vi "simple_continous_read.vi"() -> ()   [LabVIEW 2013]
doc: "This example illustrate how to use some of the VI included in the OpenBCI toolbox"
uses:
  Comm Protocol/Control Def/channel_count.ctl
panel:
  out "CH1":dbl[](graph)
  in  "channel_count(8)":T1
  out "sample count":dbl[](graph)
  in  "stop":bool
  out "EEG Waveform Channels 1 - 8":dbl[][](graph)
  out "Console":string
  in  "COM port":refnum<visa-resource-name>
  # "Instructions:\nBefore running the VI\n1. Select the COM port for the OpenBCI receiver\n2. Select the number of channels in your board\n3. Run the VI\n4. The Device initial response is shown in the Console textbox  \n5. Click on \"Stop\" to stop the EEG acquisition"
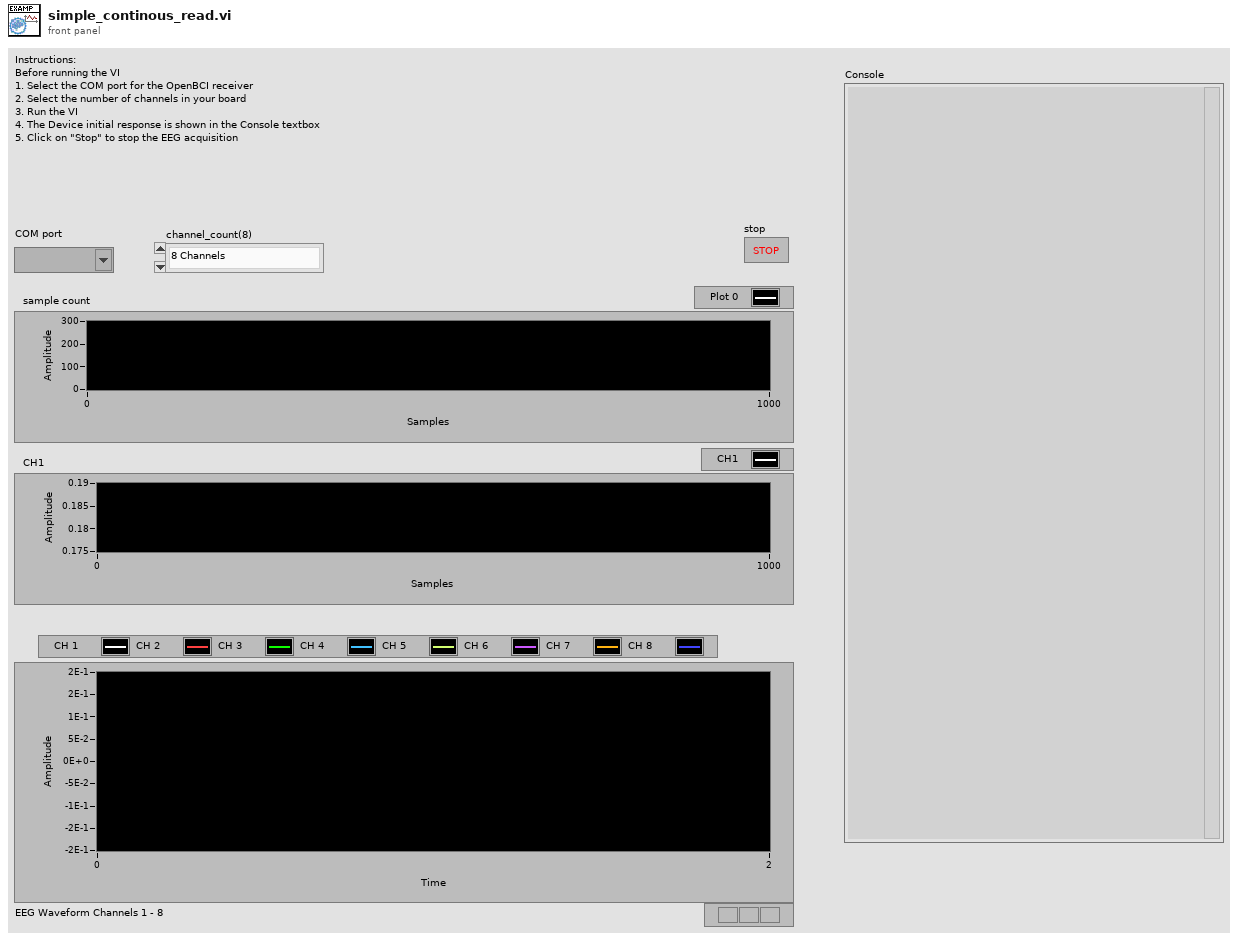
[diagram p1: front panel]
types:
  T1 = typedef "channel_count.ctl" = enum16{"8 Channels", "16 Channels"}
  T2 = typedef "openbci_device.ctl" = cluster{"COM port":refnum<visa-resource-name>, "n_ch (8)":T1, "delay_tx":u32}
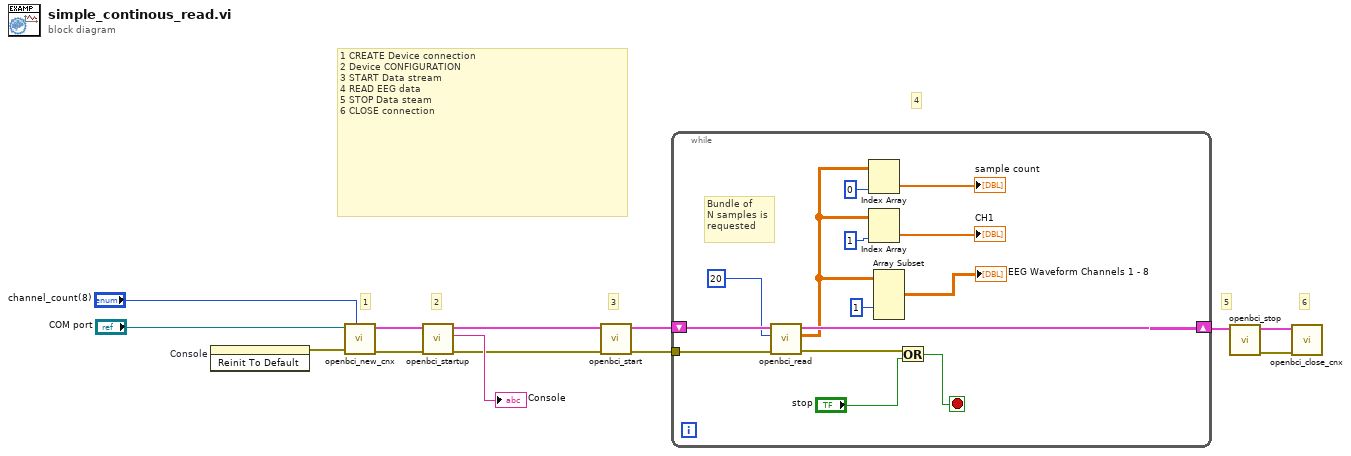
[diagram p0: block diagram]
diagram:
  # "1"
  # "4"
  # "6"
  # "5"
  # "3"
  # "2"
  # "1 CREATE Device connection\n2 Device CONFIGURATION\n3 START Data stream \n4 READ EEG data\n5 STOP Data steam\n6 CLOSE connection"
  n1 = invoke on="Console" class="Str" method="Reinit To Default"() -> (error out=w1:errorcluster)  [unwired: 3 in, 2 out]
  n2 = call "openbci_new_cnx.vi"("channel_count(8)"="channel_count(8)", "error in (no error)"=w1, "COM port"="COM port") -> ("error out"=w8:errorcluster, "OBCI dev out"=w5:T2)  [unwired: 7 in]
  n3 = call "openbci_startup.vi"("error in"=w8, "OBCI dev in"=w5) -> ("error out"=w9:errorcluster, "start_up_string"=→"Console":string, "OBCI dev out"=w4:T2)  [unwired: 7 in]
  n4 = call "openbci_start.vi"("error in (no error)"=w9, "OBCI dev in"=w4) -> ("error out"=w10:errorcluster, "OBCI dev out"=w11:T2)  [unwired: 8 in]
  n5 = while {
    shift-right: [w26] -> w12
    shift-left: w11 -> [w27]
    tunnel: w10 -> [w24]
    stop <- w22 stop-if-true
    # "Bundle of \nN samples is\nrequested"
    n6 = call "openbci_read.vi"("error in"=w24, "N samples (2)"=20, "OBCI dev in"=w27) -> ("error out"=w23:errorcluster, "EEG data"=w14:dbl[][], "OBCI dev out"=w26:T2)  [unwired: 5 in, 1 out]
    n7 = Index Array(array=w14, index (col)=0 ("disabled index (col)")) -> (element=→"sample count":dbl[])  [unwired: 1 in]
    n8 = Index Array(array=w14, index (col)=1 ("disabled index (col)")) -> (element=→"CH1":dbl[])  [unwired: 1 in]
    n9 = Array Subset(array=w14, index (col)=1 ("index")) -> (→"EEG Waveform Channels 1 - 8":dbl[][])  [unwired: 3 in]
    n10 = Or(x=w23, y="stop") -> (x .or. y?=w22:bool)
  }
  n11 = call "openbci_stop.vi"("OBCI dev in"=w12) -> ("error out"=w2:errorcluster, "OBCI dev out"=w3:T2)  [unwired: 9 in]
  n12 = call "openbci_close_cnx.vi"("error in (no error)"=w2, "OBCI dev in"=w3) -> ()  [unwired: 9 in, 1 out]
